vi "libssh2_channel_free.vi"(8 "error in (no error)":errorcluster, 11 "channel":T1) -> (0 "error out":errorcluster)   [LabVIEW 2017, in "libssh2.lvlib"]
doc: "Release memory associated with a channel."
uses:
  libssh2.lvlib
  Channel Refnum.ctl
  Global Settings.vi
  Read Session Refnum.vi
  <vilib>/Utility/semaphor.llb/Acquire Semaphore.vi
  <vilib>/Utility/semaphor.llb/Release Semaphore.vi
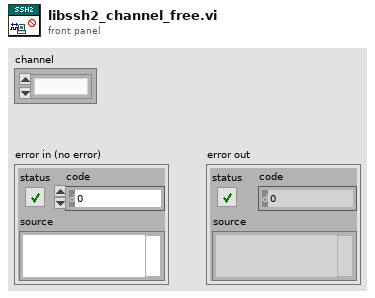
[diagram p1: front panel]
types:
  T1 = typedef "libssh2.lvlib/Channel Refnum.ctl" = refnum<k1>
  T2 = typedef "libssh2.lvlib/Session Refnum.ctl" = refnum<k1>
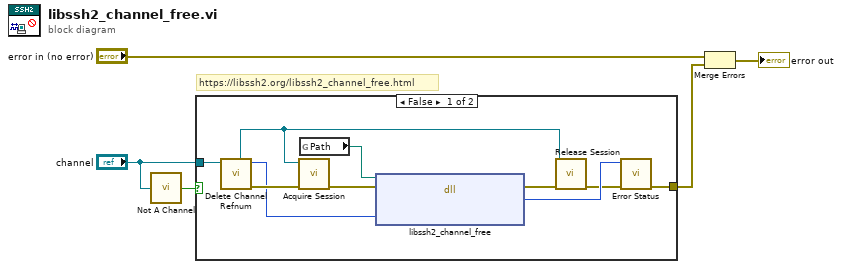
[diagram p0: block diagram]
diagram:
  # "https://libssh2.org/libssh2_channel_free.html"
  n1 = call "Not A Channel.vi"("channel"="channel") -> ("Not a Channel?"=w1:bool)
  n2 = case shown="False" w1 {
    tunnel: "channel" -> [w13 _]
    tunnel: [w10 _] -> w5
    frame False {
      n3 = call "Delete Channel Refnum.vi"("channel"=w13) -> ("error out"=w15:errorcluster, "LIBSSH2_CHANNEL*"=w14:u64, "session"=w6:T2)  [unwired: 8 in]
      n4 = call "Acquire Session.vi"("error in (no error)"=w15, "session"=w6) -> ("error out"=w7:errorcluster)  [unwired: 7 in, 2 out]
      n5 = global read "Global Settings.vi" "Path"() -> (w11:path)
      n6 = dll-call lib="?" fn="libssh2_channel_free"(path in=w11, error in=w7, "channel"=w14) -> (error out=w12:errorcluster, "return value"=w9:i32)  [unwired: 2 in, 1 out]
      n7 = call "Release Session.vi"("error in (no error)"=w12, "session"=w6) -> ("error out"=w8:errorcluster)  [unwired: 9 in]
      n8 = call "Error Status.vi"("error in (no error)"=w8, "return value"=w9) -> ("error out"=w10:errorcluster)  [unwired: 8 in, 1 out]
    }
    frame True {
    }
  }
  n9 = Merge Errors("error in (no error)", w5) -> (→"error out":errorcluster)
